vi "Sous_VI_Sceaux.vi"(8 "error in (no error)":errorcluster) -> (0 "error out":errorcluster)   [LabVIEW 2017]
uses:
  enum_bras.ctl
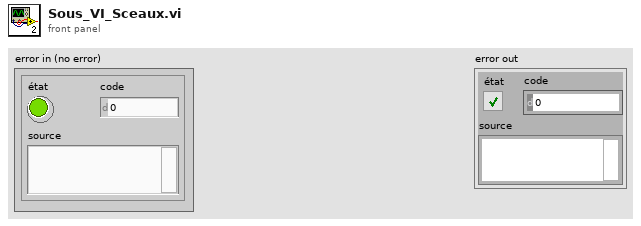
[diagram p1: front panel]
types:
  T1 = typedef "enum_bras.ctl" = enum16{"Depart Bras", "Clapet Bras", "Inactif Bras", "Seaux Bras"}
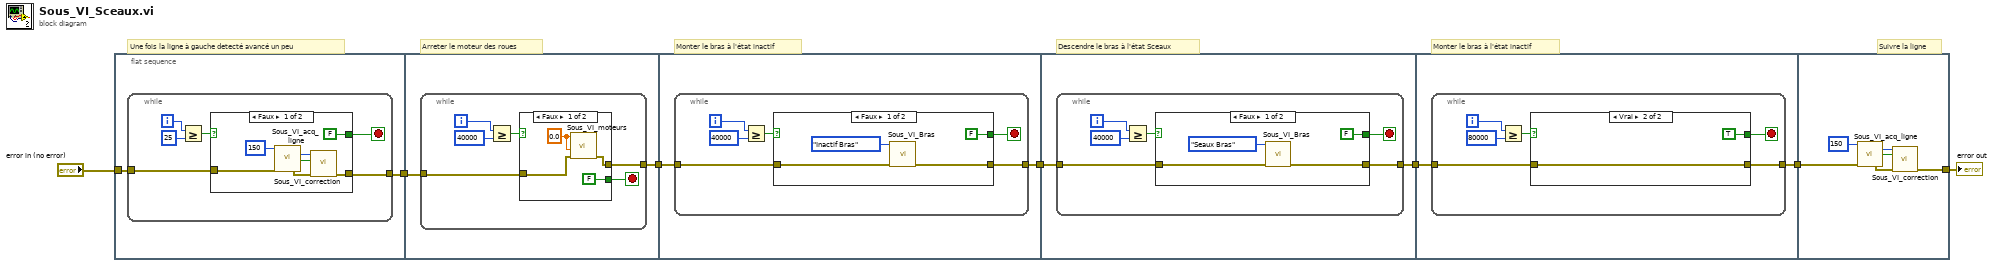
[diagram p0: block diagram]
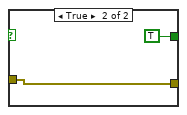
[diagram p2: hidden frame]
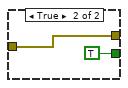
[diagram p3: hidden frame]
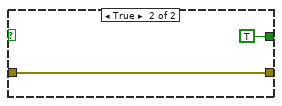
[diagram p4: hidden frame]
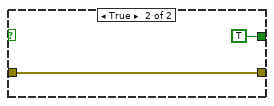
[diagram p5: hidden frame]
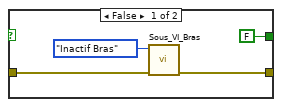
[diagram p6: hidden frame]
diagram:
  # "Suivre la ligne"
  # "Monter le bras à l'état inactif"
  # "Descendre le bras à l'état Sceaux"
  # "Monter le bras à l'état inactif"
  # "Arreter le moteur des roues"
  # "Une fois la ligne à gauche detecté avancé un peu"
  n1 = flat-sequence {
    tunnel: "error in (no error)" -> [w9]
    tunnel: [w8] -> w6
    tunnel: w6 -> [w26]
    tunnel: [w25] -> w5
    tunnel: w5 -> [w40]
    tunnel: [w39] -> w4
    tunnel: w4 -> [w54]
    tunnel: [w53] -> w3
    tunnel: w3 -> [w68]
    tunnel: [w67] -> w2
    tunnel: w2 -> [w83]
    tunnel: [w81] -> w1
    frame #0 {
      n2 = while {
        tunnel: w9 -> [w11]
        tunnel: [w10] -> w8
        i -> [w12]
        stop <- w14 stop-if-true
        n3 = Greater Or Equal?(x=w12, y=25) -> (x >= y?=w15:bool)
        n4 = case shown="Faux" w15 {
          tunnel: [FALSE TRUE] -> w14
          tunnel: w11 -> [w18 w23]
          tunnel: [w16 w23] -> w10
          frame False {
            n5 = call "Sous_VI_acq_ligne.vi"("Seuil"=150, "error in (no error)"=w18) -> ("Décalage"=w21:u32, "G/D ?"=w19:bool, "error out"=w17:errorcluster)  [unwired: 8 in, 3 out]
            n6 = call "Sous_VI_correction.vi"("error in (no error)"=w17, "G/D ?"=w19, "Décalage"=w21) -> ("error out"=w16:errorcluster)  [unwired: 8 in]
          }
          frame True {
          }
        }
      }
    }
    frame #1 {
      n7 = while {
        tunnel: w26 -> [w28]
        tunnel: [w27] -> w25
        i -> [w29]
        stop <- w31 stop-if-true
        n8 = Greater Or Equal?(x=w29, y=40000) -> (x >= y?=w32:bool)
        n9 = case shown="Faux" w32 {
          tunnel: [FALSE TRUE] -> w31
          tunnel: w28 -> [w34 w37]
          tunnel: [w33 w37] -> w27
          frame False {
            w35 = 0.0 ("Moteur Gauche")
            n10 = call "Sous_VI_moteurs.vi"("error in (no error)"=w34, "Moteur Droit"=w35, "Moteur Gauche"=w35) -> ("error out"=w33:errorcluster)  [unwired: 8 in]
          }
          frame True {
          }
        }
      }
    }
    frame #2 {
      n11 = while {
        tunnel: w40 -> [w42]
        tunnel: [w41] -> w39
        i -> [w43]
        stop <- w45 stop-if-true
        n12 = Greater Or Equal?(x=w43, y=40000) -> (x >= y?=w46:bool)
        n13 = case shown="Faux" w46 {
          tunnel: [FALSE TRUE] -> w45
          tunnel: w42 -> [w48 w51]
          tunnel: [w47 w51] -> w41
          frame False {
            n14 = call "Sous_VI_Bras.vi"("error in (no error)"=w48, "Enum bras"=enum_bras."Inactif Bras") -> ("error out"=w47:errorcluster)  [unwired: 9 in]
          }
          frame True {
          }
        }
      }
    }
    frame #3 {
      n15 = while {
        tunnel: w54 -> [w56]
        tunnel: [w55] -> w53
        i -> [w57]
        stop <- w59 stop-if-true
        n16 = Greater Or Equal?(x=w57, y=40000) -> (x >= y?=w60:bool)
        n17 = case shown="Faux" w60 {
          tunnel: [FALSE TRUE] -> w59
          tunnel: w56 -> [w62 w65]
          tunnel: [w61 w65] -> w55
          frame False {
            n18 = call "Sous_VI_Bras.vi"("error in (no error)"=w62, "Enum bras"=enum_bras."Seaux Bras") -> ("error out"=w61:errorcluster)  [unwired: 9 in]
          }
          frame True {
          }
        }
      }
    }
    frame #4 {
      n19 = while {
        tunnel: w68 -> [w70]
        tunnel: [w69] -> w67
        i -> [w71]
        stop <- w73 stop-if-true
        n20 = Greater Or Equal?(x=w71, y=80000) -> (x >= y?=w74:bool)
        n21 = case shown="Vrai" w74 {
          tunnel: [FALSE TRUE] -> w73
          tunnel: w70 -> [w76 w79]
          tunnel: [w75 w79] -> w69
          frame False {
            n22 = call "Sous_VI_Bras.vi"("error in (no error)"=w76, "Enum bras"=enum_bras."Inactif Bras") -> ("error out"=w75:errorcluster)  [unwired: 9 in]
          }
          frame True {
          }
        }
      }
    }
    frame #5 {
      n23 = call "Sous_VI_acq_ligne.vi"("Seuil"=150, "error in (no error)"=w83) -> ("Décalage"=w86:u32, "G/D ?"=w84:bool, "error out"=w82:errorcluster)  [unwired: 8 in, 3 out]
      n24 = call "Sous_VI_correction.vi"("error in (no error)"=w82, "G/D ?"=w84, "Décalage"=w86) -> ("error out"=w81:errorcluster)  [unwired: 8 in]
    }
  }
  "error out" <- w1
